vi "PIDController_AtSetpoint.vi"(11 "in PID_CONTROLLER":T1={"Kp"=0.0, "Ki"=0.0, "Kd"=0.0, "Period"=0.0, "Max_Integral"=0.0, "Min_Integral"=0.0, "Max_Input"=0.0, "Min_Input"=0.0, "Continuous"=FALSE, "PositionError"=0.0, "VelocityError"=0.0, "PrevError"=0.0, "Total_Integral"=0.0, "PositionTolerance"=0.0, "VelocityTolerance"=0.0, "SetPoint"=0.0, "Kf"=0.0, "Prev_Deriv"=0.0, "Prev_Deriv 2"=0.0, "DerivativeFilter"=FALSE, "Min_Output"=-9.99e+35, "Max_Output"=9.9e+35, "Prev_F_P"=0.0, "Prev_F_P_2"=0.0, "AntiWindupActive"=FALSE, "Measurement"=0.0, "IntegralZone"=9.9e+30} {"IntegralZone" format="%16_6e"; "Measurement" format="%16_6e"; "Prev_F_P_2" format="%16_6e"; "Prev_F_P" format="%16_6e"; "Max_Output" format="%16_6e"; "Min_Output" format="%16_6e"; "Prev_Deriv 2" format="%16_6e"; "Prev_Deriv" format="%16_6e"; "Kf" format="%16_6e"; "SetPoint" format="%16_6e"; "VelocityTolerance" format="%16_6e"; "PositionTolerance" format="%16_6e"; "Total_Integral" format="%16_6e"; "PrevError" format="%16_6e"; "VelocityError" format="%16_6e"; "PositionError" format="%16_6e"; "Min_Input" format="%16_6e"; "Max_Input" format="%16_6e"; "Min_Integral" format="%16_6e"; "Max_Integral" format="%16_6e"; "Period" format="%16_6e"; "Kd" format="%16_6e"; "Ki" format="%16_6e"; "Kp" format="%16_6e"}) -> (3 "AtSetpoint":bool)   [LabVIEW 2019, in "Trajectory_Library.lvlib"]
doc: "Returns true if the error is within the percentage of the total input range, determined by SetTolerance. This asssumes that the maximum and minimum input were set using SetInput.\n \nThis will return false until at least one input value has been computed.\n\nThis uses the error values from the most recently called calculate routine. It should be called after calling the calculate routine.\n \nInputs:\n - PID_Controller -- PID_Controller data cluster\n\nOutputs:\n - AtSetpoint -- Whether the error is within the acceptable bounds."
uses:
  Trajectory_Library.lvlib
  TypeDef/PID_CONTROLLER.ctl
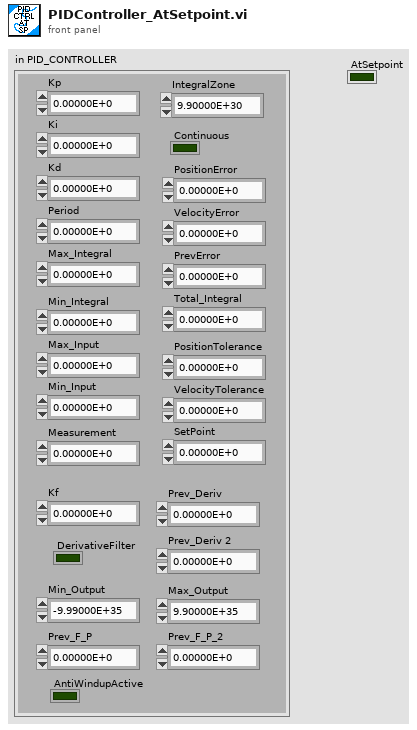
[diagram p1: front panel]
types:
  T1 = typedef "Trajectory_Library.lvlib/PID_CONTROLLER.ctl" = cluster{"Kp":dbl, "Ki":dbl, "Kd":dbl, "Period":dbl, "Max_Integral":dbl, "Min_Integral":dbl, "Max_Input":dbl, "Min_Input":dbl, "Continuous":bool, "PositionError":dbl, "VelocityError":dbl, "PrevError":dbl, "Total_Integral":dbl, "PositionTolerance":dbl, "VelocityTolerance":dbl, "SetPoint":dbl, "Kf":dbl, "Prev_Deriv":dbl, "Prev_Deriv 2":dbl, "DerivativeFilter":bool, "Min_Output":dbl, "Max_Output":dbl, "Prev_F_P":dbl, "Prev_F_P_2":dbl, "AntiWindupActive":bool, "Measurement":dbl, "IntegralZone":dbl}
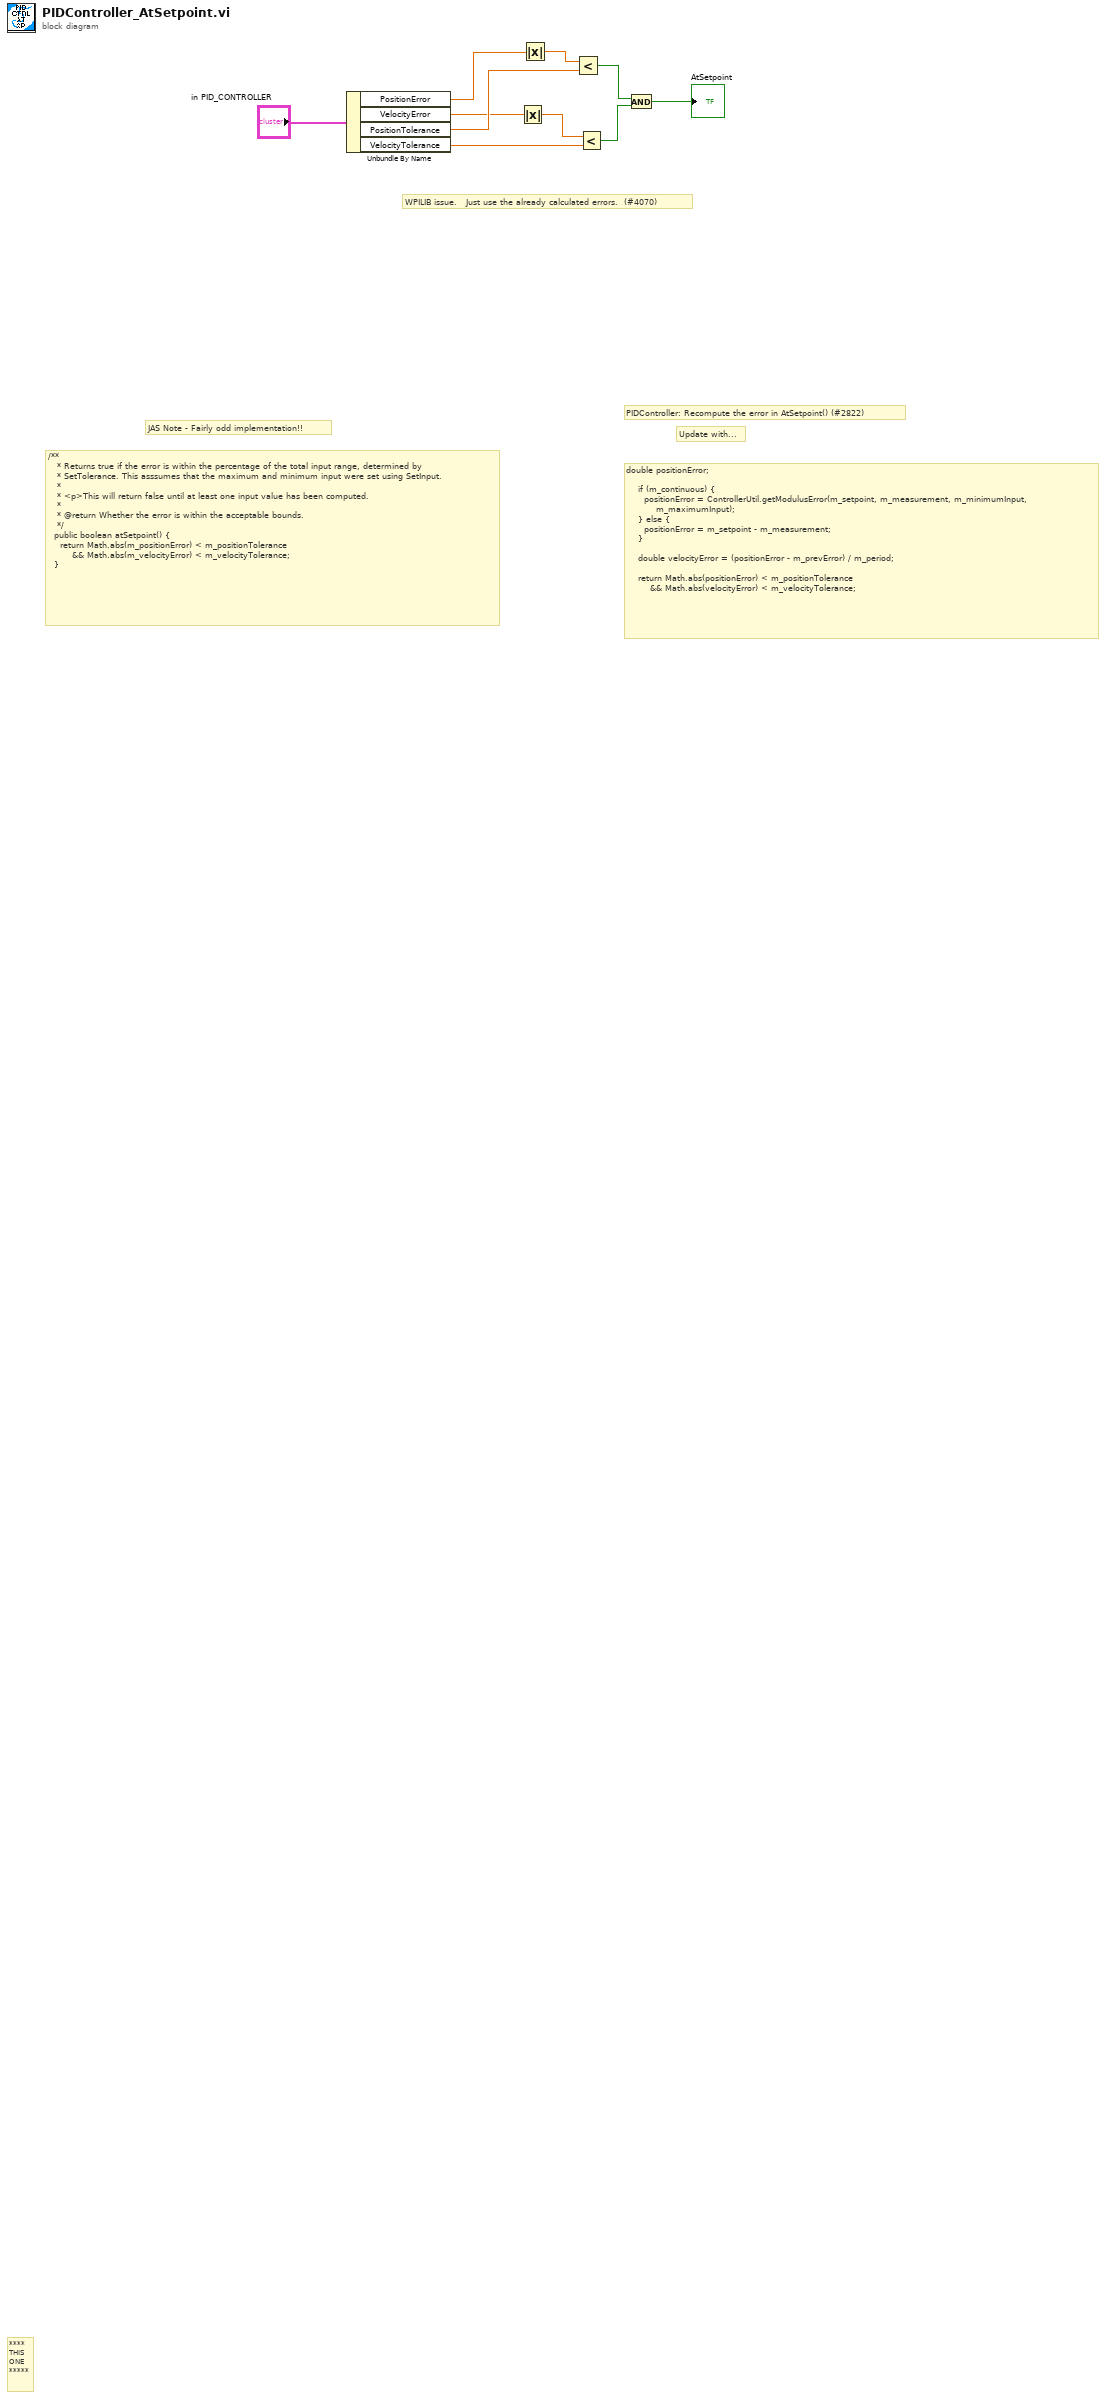
[diagram p0: block diagram]
diagram:
  # "WPILIB issue.   Just use the already calculated errors.  (#4070)"
  # "Update with..."
  # "double positionError;\n\n    if (m_continuous) {\n      positionError = ControllerUtil.getModulusError(m_setpoint, m_measurement, m_minimumInput,\n          m_maximumInput);\n    } else {\n      positionError = m_setpoint - m_measurement;\n    }\n\n    double velocityError = (positionError - m_prevError) / m_period;\n\n    return Math.abs(positionError) < m_positionTolerance\n        && Math.abs(velocityError) < m_velocityTolerance;"
  # "PIDController: Recompute the error in AtSetpoint() (#2822)"
  # "JAS Note - Fairly odd implementation!!"
  # "/**\n   * Returns true if the error is within the percentage of the total input range, determined by\n   * SetTolerance. This asssumes that the maximum and minimum input were set using SetInput.\n   *\n   * <p>This will return false until at least one input value has been computed.\n   *\n   * @return Whether the error is within the acceptable bounds.\n   */\n  public boolean atSetpoint() {\n    return Math.abs(m_positionError) < m_positionTolerance\n        && Math.abs(m_velocityError) < m_velocityTolerance;\n  }"
  # "****\nTHIS\nONE\n*****"
  n1 = Unbundle By Name("in PID_CONTROLLER") -> ("PositionError"=w2:dbl, "VelocityError"=w1:dbl, "PositionTolerance"=w5:dbl, "VelocityTolerance"=w4:dbl)
  n2 = Absolute Value(x=w1) -> (abs(x)=w9:dbl)
  n3 = Absolute Value(x=w2) -> (abs(x)=w10:dbl)
  n4 = Less?(x=w10, y=w5) -> (x < y?=w8:bool)
  n5 = Less?(x=w9, y=w4) -> (x < y?=w7:bool)
  n6 = And(x=w8, y=w7) -> (x .and. y?=→"AtSetpoint":bool)
